vi "OwnCompat20261012_Own20261012_CreateControlFromTerminal.vi"() -> ()   [LabVIEW 2024]
panel:
  out "error out":errorcluster caption="错误输出"
  out "created_terminal_id":u32
  in  "created_terminal_id type":u32
  out "control_id":u32
  in  "control_id type":u32
  in  "terminal_id":u32
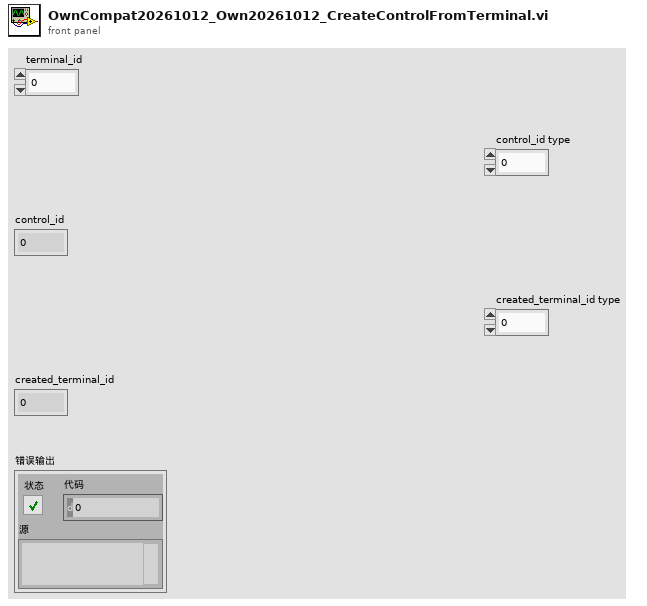
[diagram p1: front panel]
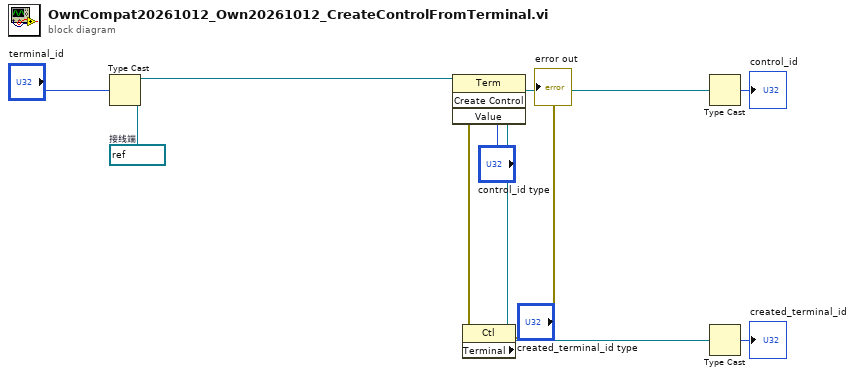
[diagram p0: block diagram]
diagram:
  w10 = refnum<vi> refnum  # 接线端
  n1 = Type Cast ("强制类型转换")(type=w10, x="terminal_id") -> (*(type *) &x=w9:refnum<vi>)
  n2 = invoke class="Term" method="Create Control"(reference=w9) -> (error out=w2:errorcluster, "Create Control"=w8:refnum<vi>)  [unwired: 3 in, 2 out]
  n3 = property on="属性节点" class="Ctl"(reference=w8, error in=w2) -> (error out=→"error out":errorcluster, "Terminal"=w5:refnum<vi>)  [unwired: 1 out]
  n4 = Type Cast ("强制类型转换")(type="control_id type", x=w8) -> (*(type *) &x=→"control_id":u32)
  n5 = Type Cast ("强制类型转换")(type="created_terminal_id type", x=w5) -> (*(type *) &x=→"created_terminal_id":u32)
